vi "RH_DCPower_Configure.vi"(6 "output terminal":tag, 7 "DCPower_Parameters":T1={"Output"=enum."DC Voltage", "Current_range"=0.0, "Current"=0.0, "Voltage_range"=0.0, "Voltage"=0.0, "Aperture_time"=0.0, "Source Delay"=0.0, "Sense"=1008} {"Source Delay" format="%.6p"; "Sense" items=["Local"=1008, "Remote"=1009]; "Aperture_time" format="%.6p"; "Current_range" format="%.6p"; "Current" format="%.6p"; "Voltage_range" format="%.6p"; "Voltage" format="%.6p"}, 8 "error in (no error)":errorcluster, 9 "trigger out?":bool, 10 "channel name":string, 11 "DCPower Session In":refnum<k15>) -> (0 "error out":errorcluster, 3 "DCPower Session Out":refnum<k15>)   [LabVIEW 2023, in "ResourceHandling.lvlib"]
doc: "Config SMU/PS channel in DC Voltage or DC Current mode, exporting Start Trigger and setting the Aperture Time"
uses:
  ResourceHandling.lvlib
  TypeDefs/RH_DCPower_Parameters.ctl
  <instrlib>/niDCPower/nidcpower.llb/niDCPower Source Mode.ctl
  <instrlib>/niDCPower/nidcpower.llb/niDCPower Output Function.ctl
  <instrlib>/niDCPower/nidcpower.llb/niDCPower Export Signal - Signal.ctl
  <instrlib>/niDCPower/nidcpower.llb/niDCPower Aperture Time Units.ctl
  <instrlib>/niDCPower/nidcpower.llb/niDCPower Disable Start Trigger With Channels.vi
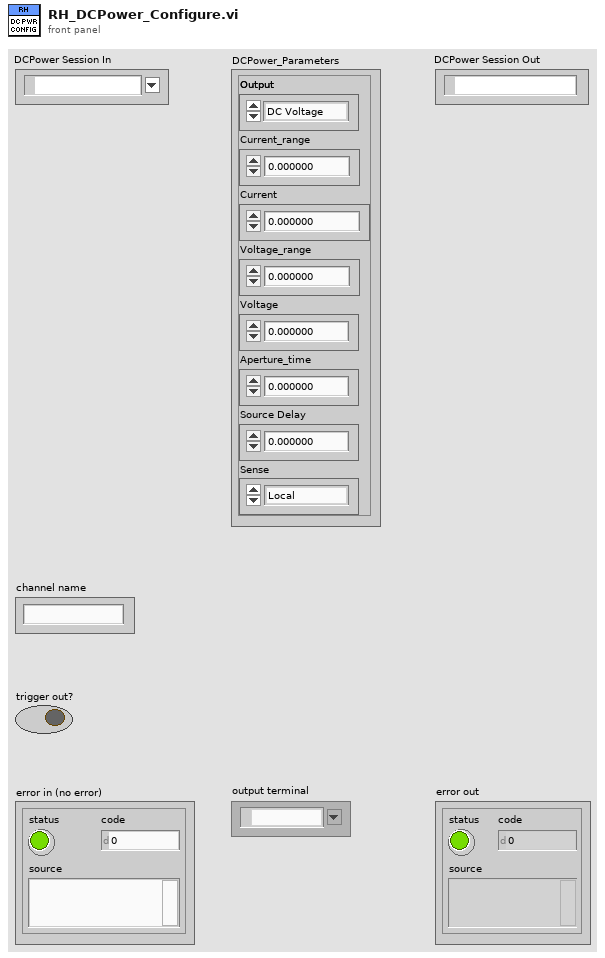
[diagram p1: front panel]
types:
  T1 = typedef "ResourceHandling.lvlib/RH_DCPower_Parameters.ctl" = cluster{"Output":enum16{"DC Voltage", "DC Current"}, "Current_range":dbl, "Current":dbl, "Voltage_range":dbl, "Voltage":dbl, "Aperture_time":dbl, "Source Delay":dbl, "Sense":i32}
  T2 = typedef "niDCPower Source Mode.ctl" = i32
  T3 = typedef "niDCPower Output Function.ctl" = i32
  T4 = typedef "niDCPower Export Signal - Signal.ctl" = i32
  T5 = typedef "niDCPower Aperture Time Units.ctl" = i32
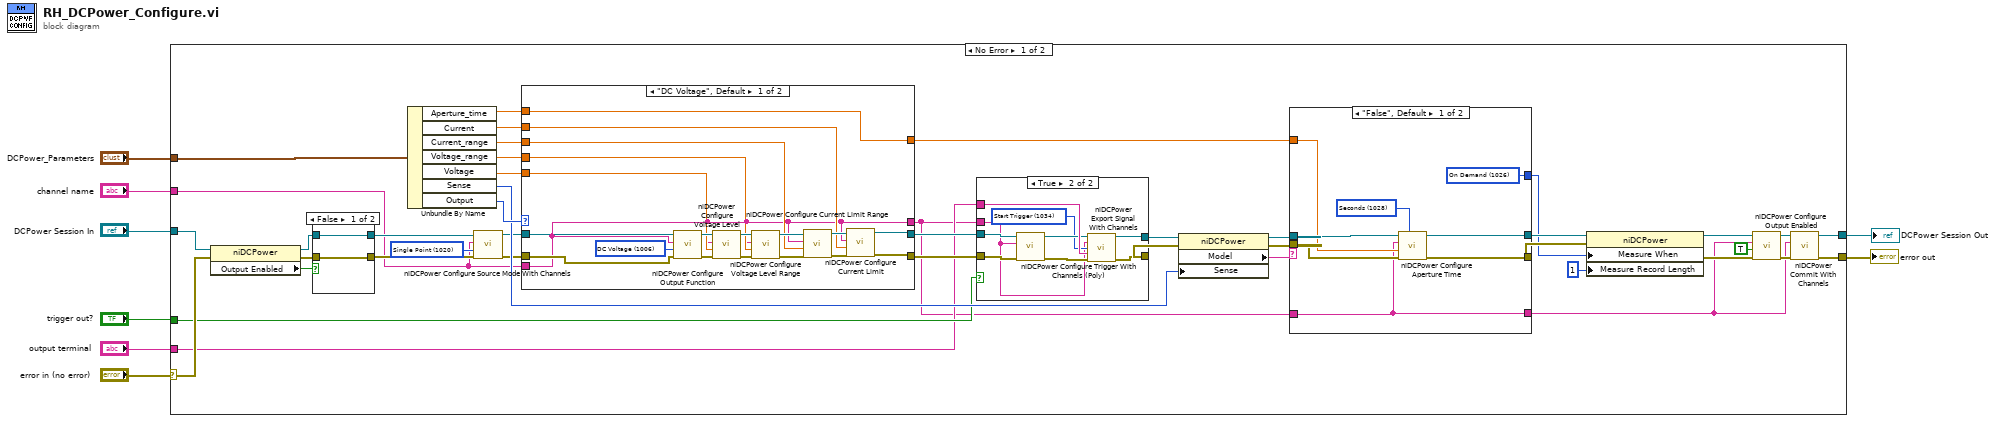
[diagram p0: block diagram]
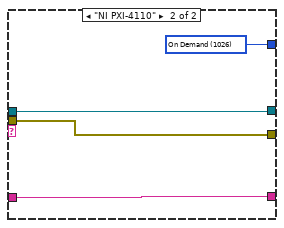
[diagram p2: hidden frame]
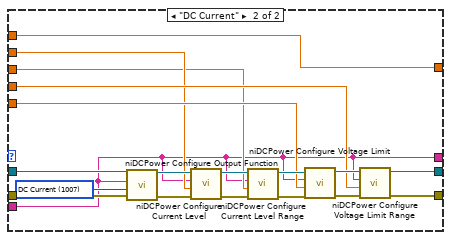
[diagram p4: hidden frame]
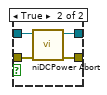
[diagram p5: hidden frame]
diagram:
  n1 = case shown="No Error" "error in (no error)" {
    selector: "error in (no error)" -> [w32 w119]
    tunnel: "DCPower_Parameters" -> [w36 _]
    tunnel: "DCPower Session In" -> [w35 w118]
    tunnel: [w34 w118] -> w1
    tunnel: [w33 w119] -> w7
    tunnel: "channel name" -> [w11 _]
    tunnel: "trigger out?" -> [w20 _]
    tunnel: "output terminal" -> [w19 _]
    frame No Error {
      w25 = T2 1020 items=["Single Point"=1020, "Sequence"=1021] ("source mode")
      n2 = property class="niDCPower"(reference=w35, error in=w32) -> (reference out=w49:refnum<k15>, error out=w50:errorcluster, "Output Enabled"=w48:bool)
      n3 = case shown="False" w48 {
        tunnel: w49 -> [w113 w117]
        tunnel: w50 -> [w112 w116]
        tunnel: [w113 w115] -> w29
        tunnel: [w112 w114] -> w27
        frame False {
        }
        frame True {
          n4 = call <instrlib>:"niDCPower Abort.vi"("error in (no error)"=w116, "instrument handle"=w117) -> ("error out"=w114:errorcluster, "instrument handle out"=w115:refnum<k15>)  [unwired: 8 in]
        }
      }
      n5 = Unbundle By Name(w36) -> ("Aperture_time"=w41:dbl, "Current"=w42:dbl, "Current_range"=w43:dbl, "Voltage_range"=w44:dbl, "Voltage"=w45:dbl, "Sense"=w30:i32, "Output"=w31:enum16{"DC Voltage", "DC Current"})
      n6 = call <instrlib>:"niDCPower Configure Source Mode With Channels.vi"("error in (no error)"=w27, "source mode"=w25, "channel name"=w11, "instrument handle"=w29) -> ("error out"=w26:errorcluster, "instrument handle out"=w28:refnum<k15>)  [unwired: 6 in]
      n7 = case shown="\"DC Voltage\", Default" w31 {
        tunnel: w26 -> [w83 w103]
        tunnel: w28 -> [w84 w102]
        tunnel: [w77 w98] -> w24
        tunnel: [w76 w97] -> w22
        tunnel: w45 -> [w87 w99]
        tunnel: w44 -> [w86 w100]
        tunnel: w43 -> [w80 w94]
        tunnel: w42 -> [w75 w95]
        tunnel: w41 -> [w85 w96]
        tunnel: [w85 w96] -> w37
        tunnel: w11 -> [w74 w93]
        tunnel: [w74 w93] -> w13
        frame "DC Voltage", Default {
          w88 = T3 1006 items=["DC Voltage"=1006, "DC Current"=1007, "Pulse Voltage"=1049, "Pulse Current"=1050] ("output function")
          n8 = call <instrlib>:"niDCPower Configure Output Function.vi"("error in (no error)"=w83, "output function"=w88, "channel name"=w74, "instrument handle"=w84) -> ("error out"=w90:errorcluster, "instrument handle out"=w89:refnum<k15>)  [unwired: 6 in]
          n9 = call <instrlib>:"niDCPower Configure Voltage Level.vi"("error in (no error)"=w90, "voltage level"=w87, "channel name"=w74, "instrument handle"=w89) -> ("error out"=w92:errorcluster, "instrument handle out"=w91:refnum<k15>)  [unwired: 6 in]
          n10 = call <instrlib>:"niDCPower Configure Voltage Level Range.vi"("error in (no error)"=w92, "voltage level range"=w86, "channel name"=w74, "instrument handle"=w91) -> ("error out"=w82:errorcluster, "instrument handle out"=w81:refnum<k15>)  [unwired: 6 in]
          n11 = call <instrlib>:"niDCPower Configure Current Limit Range.vi"("error in (no error)"=w82, "current limit range"=w80, "channel name"=w74, "instrument handle"=w81) -> ("error out"=w79:errorcluster, "instrument handle out"=w78:refnum<k15>)  [unwired: 6 in]
          n12 = call <instrlib>:"niDCPower Configure Current Limit.vi"("error in (no error)"=w79, "current limit"=w75, "channel name"=w74, "instrument handle"=w78) -> ("error out"=w76:errorcluster, "instrument handle out"=w77:refnum<k15>)  [unwired: 6 in]
        }
        frame "DC Current" {
          w101 = T3 1007 items=["DC Voltage"=1006, "DC Current"=1007, "Pulse Voltage"=1049, "Pulse Current"=1050] ("output function")
          n13 = call <instrlib>:"niDCPower Configure Output Function.vi"("error in (no error)"=w103, "output function"=w101, "channel name"=w93, "instrument handle"=w102) -> ("error out"=w104:errorcluster, "instrument handle out"=w105:refnum<k15>)  [unwired: 6 in]
          n14 = call <instrlib>:"niDCPower Configure Current Level.vi"("error in (no error)"=w104, "current level"=w95, "channel name"=w93, "instrument handle"=w105) -> ("error out"=w111:errorcluster, "instrument handle out"=w110:refnum<k15>)  [unwired: 6 in]
          n15 = call <instrlib>:"niDCPower Configure Current Level Range.vi"("error in (no error)"=w111, "current level range"=w94, "channel name"=w93, "instrument handle"=w110) -> ("error out"=w109:errorcluster, "instrument handle out"=w108:refnum<k15>)  [unwired: 6 in]
          n16 = call <instrlib>:"niDCPower Configure Voltage Limit.vi"("error in (no error)"=w109, "voltage limit"=w99, "channel name"=w93, "instrument handle"=w108) -> ("error out"=w107:errorcluster, "instrument handle out"=w106:refnum<k15>)  [unwired: 6 in]
          n17 = call <instrlib>:"niDCPower Configure Voltage Limit Range.vi"("error in (no error)"=w107, "voltage limit range"=w100, "channel name"=w93, "instrument handle"=w106) -> ("error out"=w97:errorcluster, "instrument handle out"=w98:refnum<k15>)  [unwired: 6 in]
        }
      }
      n18 = case shown="True" w20 {
        tunnel: w24 -> [w64 w70]
        tunnel: [w64 w73] -> w23
        tunnel: w22 -> [w63 w68]
        tunnel: [w63 w72] -> w21
        tunnel: w19 -> [_ w71]
        tunnel: w13 -> [_ w65]
        frame False {
        }
        frame True {
          w66 = T4 1034 items=["Source Complete Event"=1030, "Measure Complete Event"=1031, "Sequence Iteration Complete Event"=1032, "Sequence Engine Done Event"=1033, "Pulse Complete Event"=1051, "Ready For Pulse Trigger Event"=1052, "Start Trigger"=1034, "Source Trigger"=1035, "Measure Trigger"=1036, "Sequence Advance Trigger"=1037, "Pulse Trigger"=1053] ("signal")
          n19 = call-poly <instrlib>:"niDCPower Configure Trigger With Channels (Poly).vi"("error in (no error)"=w68, "channel name"=w65, "instrument handle"=w70) -> ("error out"=w67:errorcluster, "instrument handle out"=w69:refnum<k15>)  [unwired: 7 in]
          n20 = call <instrlib>:"niDCPower Export Signal With Channels.vi"("instrument handle"=w69, "channel name"=w65, "signal"=w66, "output terminal"=w71, "error in (no error)"=w67) -> ("instrument handle out"=w73:refnum<k15>, "error out"=w72:errorcluster)  [unwired: 9 in]
        }
      }
      n21 = property class="niDCPower"(reference=w23, error in=w21, "Sense"=w30) -> (reference out=w39:refnum<k15>, error out=w38:errorcluster, "Model"=w40:string)
      n22 = case shown="\"False\", Default" w40 {
        tunnel: w39 -> [w58 w62]
        tunnel: w38 -> [w57 w61]
        tunnel: [w56 w61] -> w17
        tunnel: [w55 w62] -> w18
        tunnel: w37 -> [w54 _]
        tunnel: w13 -> [w52 w60]
        tunnel: [w52 w60] -> w12
        tunnel: [w51 w59] -> w14
        frame "False", Default {
          w51 = 1026 items=["Automatically after Source Complete"=1025, "On Demand"=1026, "On Measure Trigger"=1027] ("Measurement:Advanced:Measure When")
          w53 = T5 1028 items=["Seconds"=1028, "Powerline Cycles"=1029] ("aperture time units")
          n23 = call <instrlib>:"niDCPower Configure Aperture Time.vi"("aperture time units"=w53, "error in (no error)"=w57, "aperture time"=w54, "channel name"=w52, "instrument handle"=w58) -> ("error out"=w56:errorcluster, "instrument handle out"=w55:refnum<k15>)  [unwired: 5 in]
        }
        frame "NI PXI-4110" {
          w59 = 1026 items=["Automatically after Source Complete"=1025, "On Demand"=1026, "On Measure Trigger"=1027] ("Measurement:Advanced:Measure When")
        }
      }
      n24 = property class="niDCPower"(reference=w18, error in=w17, "Measure When"=w14, "Measure Record Length"=1 ("Measurement:Measure Record Length")) -> (reference out=w15:refnum<k15>, error out=w16:errorcluster)
      n25 = call <instrlib>:"niDCPower Configure Output Enabled.vi"("error in (no error)"=w16, "output enabled"=TRUE, "channel name"=w12, "instrument handle"=w15) -> ("error out"=w47:errorcluster, "instrument handle out"=w46:refnum<k15>)  [unwired: 6 in]
      n26 = call <instrlib>:"niDCPower Commit With Channels.vi"("error in (no error)"=w47, "channel name"=w12, "instrument handle"=w46) -> ("error out"=w33:errorcluster, "instrument handle out"=w34:refnum<k15>)  [unwired: 7 in]
    }
    frame Error {
    }
  }
  "error out" <- w7
  "DCPower Session Out" <- w1
